vi "Instructions_segments EPC.vi"(0 "Numéro de segment":i8) -> (4 "chaîne $":string, 6 "chaîne s":string, 8 "chaîne d":string, 10 "chaîne p":string, 15 "chaîne o":string)   [LabVIEW 2022 SP3]
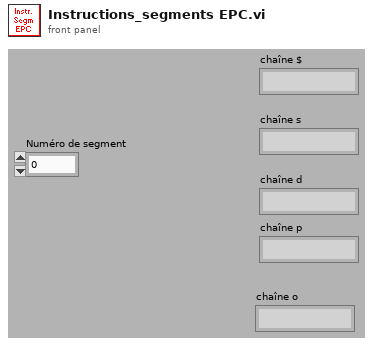
[diagram p1: front panel]
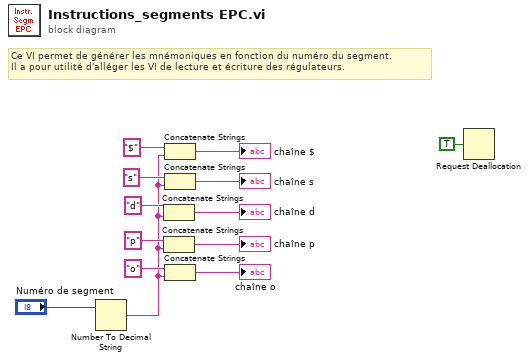
[diagram p0: block diagram]
diagram:
  # "Ce VI permet de générer les mnémoniques en fonction du numéro du segment.\nIl a pour utilité d'alléger les VI de lecture et écriture des régulateurs."
  n1 = Number To Decimal String(number="Numéro de segment") -> (decimal integer string=w1:string)  [unwired: 1 in]
  n2 = Concatenate Strings("d", w1) -> (→"chaîne d":string)
  n3 = Concatenate Strings("p", w1) -> (→"chaîne p":string)
  n4 = Concatenate Strings("$", w1) -> (→"chaîne $":string)
  n5 = Concatenate Strings("s", w1) -> (→"chaîne s":string)
  n6 = Concatenate Strings("o", w1) -> (→"chaîne o":string)
  n7 = Request Deallocation(TRUE ("flag")) -> ()
